vi "RDV-addDataToMapFromFile.vi"(5 "Add mod":string, 7 "Folder Path":path=path "C:/projects/Universitet/Master/data/Real Test - First libreVNA test with calibration file/Converted Data", 8 "error in (no error)":errorcluster, 11 "RDV-Reflection_Data_viewer in":refnum<class "RDV-Reflection_Data_viewer.lvclass">) -> (0 "error out":errorcluster, 2 "Keys":string[](array[string]), 3 "RDV-Reflection_Data_viewer out":refnum<class "RDV-Reflection_Data_viewer.lvclass">)   [LabVIEW 2020, in "RDV-Reflection_Data_viewer.lvclass"]
doc: "Reads every common-format file in a folder and adds the data to the viewer's map, with keys from the file names and Add mod. Returns the keys."
uses:
  RDV-Reflection_Data_viewer.lvclass
  Reflector/RFH-Reflection_File_Handler.lvlib
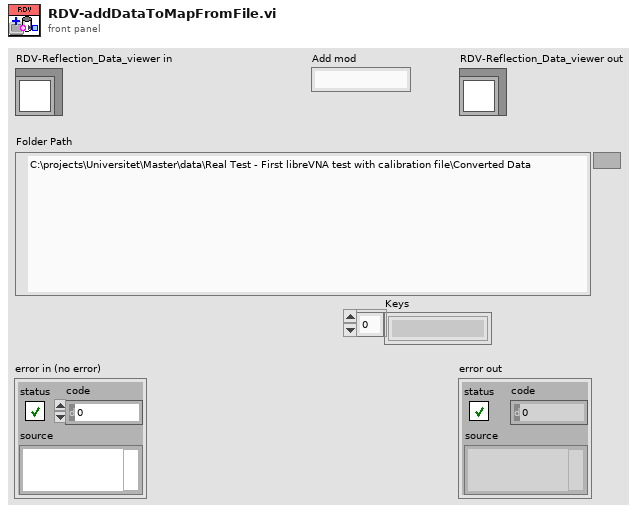
[diagram p1: front panel]
types:
  T1 = typedef "RFH-Reflection_File_Handler.lvlib/RFH-common_data_format.ctl" = cluster{"Frequency":dbl[], "Reflection'":dbl[], "Reflection''":dbl[], "Permativity'":dbl[], "Permativity''":dbl[], "Conductivity":dbl[], "Loss Tangent":dbl[], "Resistance":dbl[], "Reactance":dbl[]}
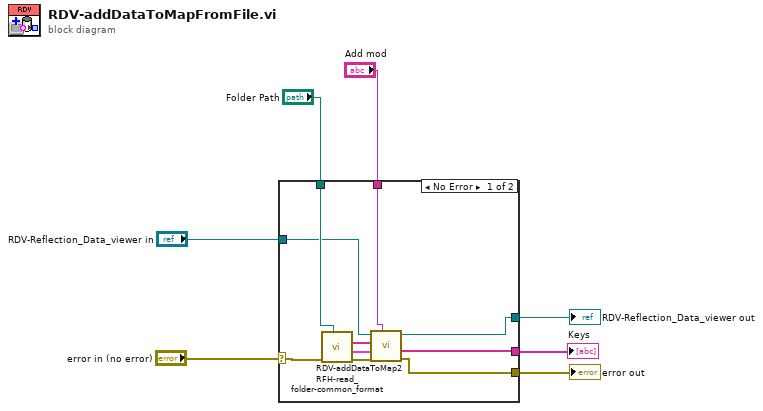
[diagram p0: block diagram]
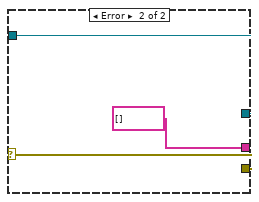
[diagram p2: hidden frame]
diagram:
  n1 = case shown="No Error" "error in (no error)" {
    selector: "error in (no error)" -> [w16 w20]
    tunnel: [w8 w20] -> w6
    tunnel: [w9 w19] -> w4
    tunnel: "RDV-Reflection_Data_viewer in" -> [w15 w19]
    tunnel: "Folder Path" -> [w17 _]
    tunnel: [w10 string[] []] -> w2
    tunnel: "Add mod" -> [w11 _]
    frame No Error {
      n2 = call "RFH-read_folder-common_format.vi"("File Path"=w17, "error In"=w16) -> ("error out"=w12:errorcluster, "Data"=w13:T1[], "Names"=w14:string[])  [unwired: 7 in]
      n3 = call "RDV-addDataToMap2.vi"("Add mod"=w11, "error in (no error)"=w12, "Data"=w13, "Names"=w14, "RDV-Reflection_Data_viewer in"=w15) -> ("error out"=w8:errorcluster, "Keys"=w10:string[], "RDV-Reflection_Data_viewer out"=w9:refnum<class "RDV-Reflection_Data_viewer.lvclass">)  [unwired: 4 in]
    }
    frame Error {
    }
  }
  "error out" <- w6
  "RDV-Reflection_Data_viewer out" <- w4
  "Keys" <- w2
